vi "GetText.vi"(8 "error in":errorcluster, 11 "FPGA Module editor node in":refnum<class "FPGA Module editor node.lvclass">) -> (0 "error out":errorcluster, 1 "additional text":string, 2 "text":string, 3 "FPGA Module editor node out":refnum<class "FPGA Module editor node.lvclass">, 4 "glyph":string)   [LabVIEW 2015, in "FPGA Module editor node.lvclass"]
doc: "Use this VI to display the name of the module in the tree and to specify the desired glyph in the configuration editor."
uses:
  FPGA Module editor node.lvclass
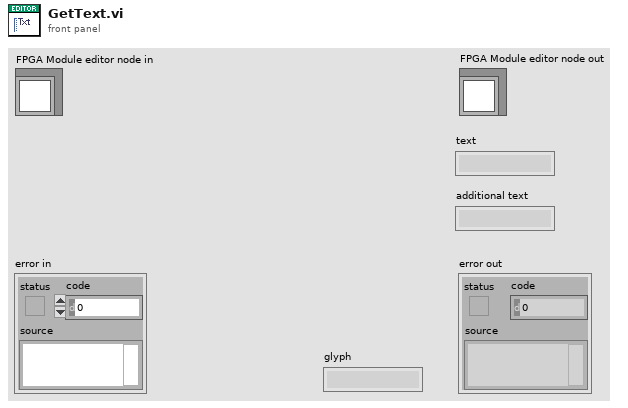
[diagram p1: front panel]
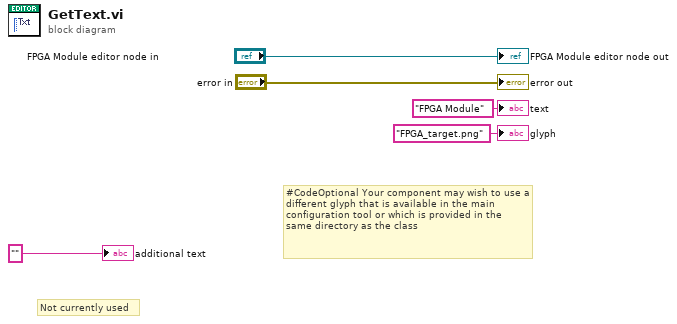
[diagram p0: block diagram]
diagram:
  # "Not currently used"
  # "#CodeOptional Your component may wish to use a different glyph that is available in the main configuration tool or which is provided in the same directory as the class"
  "error out" <- "error in"
  "FPGA Module editor node out" <- "FPGA Module editor node in"
  "text" <- "FPGA Module" ("text")
  "additional text" <- "" ("additional text")
  "glyph" <- "FPGA_target.png" ("glyph")
